vi "Load DAC Configuration.vi"(8 "error in":errorcluster, 10 "Config File refnum in":T1, 11 "DAC ADV in":refnum<class "DAC ADV.lvclass">) -> (0 "error out":errorcluster, 2 "Config File refnum out":T1, 3 "DAC ADV out":refnum<class "DAC ADV.lvclass">)   [LabVIEW 2019, in "DAC.lvlib" / "DAC ADV.lvclass"]
uses:
  DAC ADV.lvclass
  C:/Users/krio/Documents/LV_Projects/test-stand/App/DAC/DAC.lvclass
  <vilib>/Utility/config.llb/Config Data RefNum.ctl
  DAC.lvclass/DAC.ctl
  DAC ADV.lvclass/DAC ADV.ctl
  <vilib>/Utility/config.llb/Read Key (Double).vi
  DAC.lvclass
  <vilib>/Utility/config.llb/NI_LVConfig.lvlib
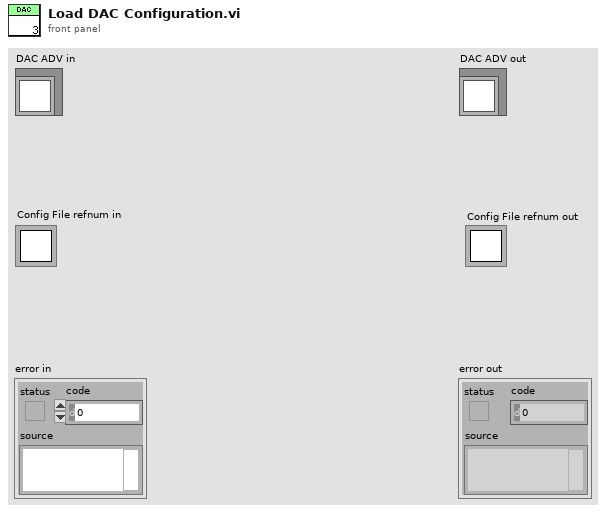
[diagram p1: front panel]
types:
  T1 = typedef "NI_LVConfig.lvlib/Config Data RefNum.ctl" = refnum<k1>
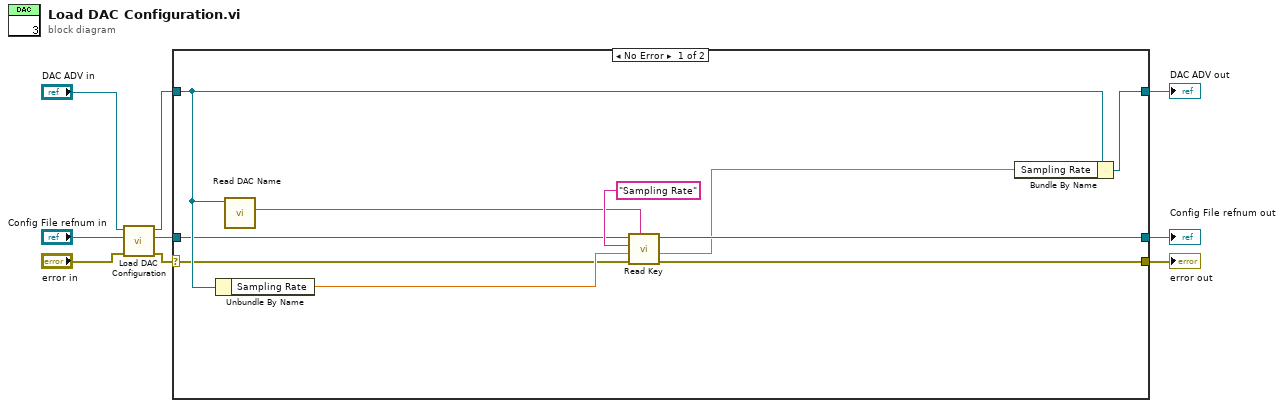
[diagram p0: block diagram]
diagram:
  n1 = call-parent "Load DAC Configuration.vi"("error in"="error in", "Config File refnum in"="Config File refnum in", "DAC in"="DAC ADV in") -> ("error out"=w4:errorcluster, "Config File refnum out"=w5:T1, "DAC out"=w6:refnum<class "DAC ADV.lvclass">)  [unwired: 6 in]
  n2 = case shown="No Error" w4 {
    selector: w4 -> [w12 w20]
    tunnel: [w18 w22] -> w3
    tunnel: w6 -> [w17 w22]
    tunnel: w5 -> [w11 w21]
    tunnel: [w14 w21] -> w2
    tunnel: [w15 w20] -> w1
    frame No Error {
      n3 = Unbundle By Name(w17) -> ("Sampling Rate"=w16:dbl)
      n4 = call "Read DAC Name.vi"("DAC in"=w17) -> ("DAC Name"=w10:string)  [unwired: 8 in, 2 out]
      n5 = call-poly <vilib>:"Read Key.vi"("section"=w10, "error in (no error)"=w12, "default value"=w16, "key"="Sampling Rate", "refnum"=w11) -> ("error out"=w15:errorcluster, "value"=w13:dbl, "refnum out"=w14:T1)  [unwired: 3 in, 1 out]
      n6 = Bundle By Name(cluster=w17, "Sampling Rate"=w13) -> (w18:refnum<class "DAC ADV.lvclass">)
    }
    frame Error {
    }
  }
  "error out" <- w1
  "DAC ADV out" <- w3
  "Config File refnum out" <- w2
